vi "RemoteVI Menu Highlight.vi"(0 "hwnd":u64, 11 "error in":errorcluster) -> (4 "found?":bool, 6 "top":i32, 8 "bottom":i32, 10 "height":i32, 12 "menu colours?":bool, 14 "submenu?":bool, 15 "error out":errorcluster)   [LabVIEW 2020, in "RemoteVI.lvlib"]
doc: "Finds the highlighted item of a LabVIEW menu window: captures hwnd (RemoteVI Capture Window.vi - PrintWindow, so it works on a menu that is invisible on the host) and looks down its middle column for pixels of the Windows highlight colour (RemoteVI System Color.vi, COLOR_HIGHLIGHT 13). LabVIEW paints the selected menu row in that colour across the whole row, with the item text in the highlight text colour on top (measured on LabVIEW 2025 ring, plot legend and shortcut menus), so the first and the last matching row are the top and bottom of the highlighted item in window pixels. found? is FALSE when no row matches - a menu nothing is highlighted in yet, or a popup that is no menu (colour picker, line width popup) - or when the capture failed (the window closed). submenu? is TRUE when the highlighted item opens a submenu: inside the band (2 px in from its top and bottom), the 18 columns that end 6 px before the right edge hold a pixel that is not the highlight colour - the submenu arrow, which LabVIEW draws there in the highlight text colour (measured on LabVIEW 2025 menu bar, shortcut and submenu menus: the band otherwise fills that strip; shortcut texts end further left). RemoteVI Hover Menus.vi presses VK_RIGHT for a hover dwell only then, because in a menu of the panels menu bar VK_RIGHT on an item without a submenu switches to the next menu bar menu (measured). menu colours? is TRUE when at least a quarter of that column has the menu background colour (COLOR_MENU 4) - every LabVIEW menu does, the colour picker does not (its background is 0xF7F7F7, measured); RemoteVI Highlight Menu Row.vi posts no probe key into a window without it, because a key posted into the colour picker spoils its next mouse click (measured: the colour was not taken). Capture errors are dropped; error in passes through unchanged. Win32 only, no VI Server call."
uses:
  RemoteVI.lvlib
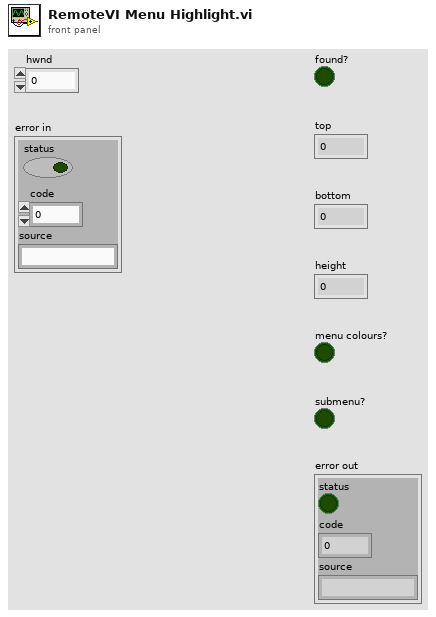
[diagram p1: front panel]
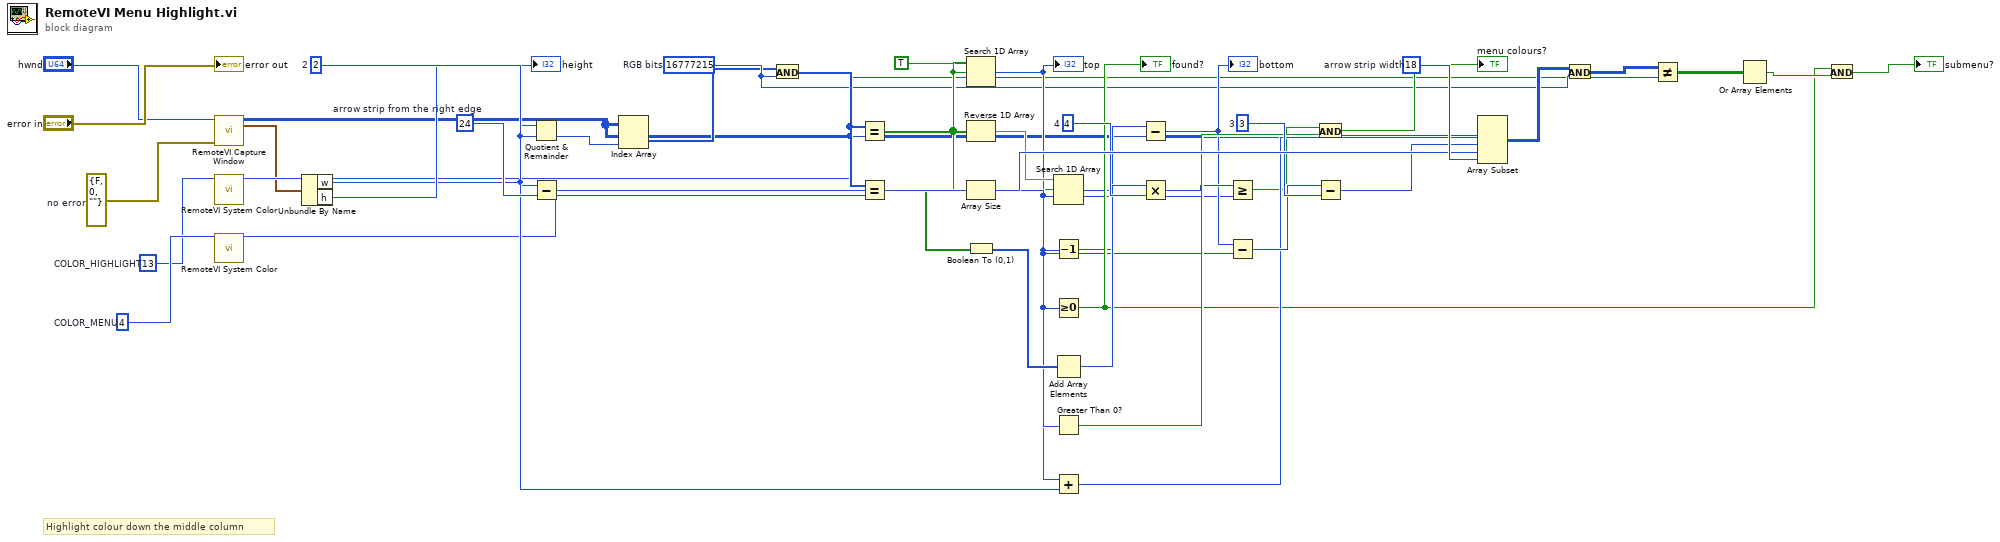
[diagram p0: block diagram]
diagram:
  w40 = 18  # arrow strip width
  w38 = 24  # arrow strip from the right edge
  w36 = 3  # 3
  w29 = 4  # 4
  w18 = TRUE
  w15 = u32 16777215  # RGB bits
  w12 = 2  # 2
  w7 = 4  # COLOR_MENU
  w6 = 13  # COLOR_HIGHLIGHT
  w3 = errorcluster {"status"=FALSE, "code"=0, "source"=""}  # no error
  # "Highlight colour down the middle column"
  n1 = call "RemoteVI Capture Window.vi"("hwnd"="hwnd", "error in"=w3) -> ("pixmap"=w4:u32[][], "rect"=w5:cluster{"x":i32, "y":i32, "w":i32, "h":i32})  [unwired: 11 in, 1 out]
  n2 = call "RemoteVI System Color.vi"("nIndex"=w6) -> ("rgb"=w8:u32)  [unwired: 14 in]
  n3 = call "RemoteVI System Color.vi"("nIndex"=w7) -> ("rgb"=w9:u32)  [unwired: 14 in]
  n4 = Unbundle By Name(w5) -> ("w"=w10:i32, "h"=→"height":i32)
  n5 = Quotient & Remainder(x=w10, y=w12) -> (floor(x/y)=w13:i32)  [unwired: 1 out]
  n6 = Subtract(x=w10, y=w38) -> (x-y=w39:i32)
  n7 = Index Array(array=w4, index (col)=w13) -> (element=w14:u32[])  [unwired: 1 in]
  n8 = And(x=w14, y=w15) -> (x .and. y?=w16:u32[])
  n9 = Equal?(x=w16, y=w8) -> (x = y?=w17:bool[])
  n10 = Equal?(x=w16, y=w9) -> (x = y?=w26:bool[])
  n11 = Search 1D Array(1D array=w17, element=w18) -> (index of element=w19:i32)  [unwired: 1 in]
  "top" <- w19
  n12 = Reverse 1D Array(array=w17) -> (reversed array=w20:bool[])
  n13 = Array Size(array=w17) -> (size(s)=w22:i32)
  n14 = Boolean To (0,1)(Boolean=w26) -> (0, 1=w27:i16[])
  n15 = Search 1D Array(1D array=w20, element=w18) -> (index of element=w21:i32)  [unwired: 1 in]
  n16 = Decrement(x=w22) -> (x-1=w23:i32)
  n17 = Greater Or Equal To 0?(x=w19) -> (x >= 0?=w25:bool)
  "found?" <- w25
  n18 = Add Array Elements(numeric array=w27) -> (sum=w28:i16)
  n19 = Greater Than 0?(x=w22) -> (x > 0?=w32:bool)
  n20 = Add(x=w19, y=w12) -> (x+y=w34:i32)
  n21 = Subtract(x=w23, y=w21) -> (x-y=w24:i32)
  "bottom" <- w24
  n22 = Multiply(x=w28, y=w29) -> (x*y=w30:i32)
  n23 = Greater Or Equal?(x=w30, y=w22) -> (x >= y?=w31:bool)
  n24 = Subtract(x=w24, y=w19) -> (x-y=w35:i32)
  n25 = And(x=w31, y=w32) -> (x .and. y?=→"menu colours?":bool)
  n26 = Subtract(x=w35, y=w36) -> (x-y=w37:i32)
  n27 = Array Subset(array=w4, index (row)=w34, length (row)=w37, index (col)=w39, length (col)=w40) -> (w41:u32[][])
  n28 = And(x=w41, y=w15) -> (x .and. y?=w42:u32[][])
  n29 = Not Equal?(x=w42, y=w8) -> (x != y?=w43:bool[][])
  n30 = Or Array Elements(Boolean array=w43) -> (logical OR=w44:bool)
  n31 = And(x=w25, y=w44) -> (x .and. y?=→"submenu?":bool)
  "error out" <- "error in"
